vi "getXMLTestSuite.vi"(9 "indent level":i32, 10 "testsuite":T1={"name"="", "errors"=0, "skipped"=0, "tests"=0, "failures"=0, "time"=-1.0, "timestamp"=timestamp(0 s since 1904-01-01), "call-chain"=[], "properties"=variant}, 11 "Test Report in":refnum<class "Test Report.lvclass">) -> (1 "testsuite (end)":string="</testsuite>", 2 "testsuite (start)":string[](array[string]), 3 "Test Report":refnum<class "Test Report.lvclass">)   [LabVIEW 2020, in "Caraya.lvlib" / "Test Report.JUnit.lvclass"]
uses:
  Test Report.JUnit.lvclass
  testsuite -- cluster.ctl
  Test Report/Test Report.lvclass
  MsgSerializer.XML/MsgSerializer.XML.lvclass
  C:/projects/caraya/src/classes/MsgSerializer/MsgSerializer.lvclass
  Test Report/Test Report.lvclass/Test Report.ctl
  MsgSerializer/MsgSerializer.lvclass/MsgSerializer.ctl
  MsgSerializer.XML/format -- enum.ctl
  MsgSerializer.XML/MsgSerializer.XML.lvclass/MsgSerializer.XML.ctl
  MsgSerializer/MsgSerializer.lvclass
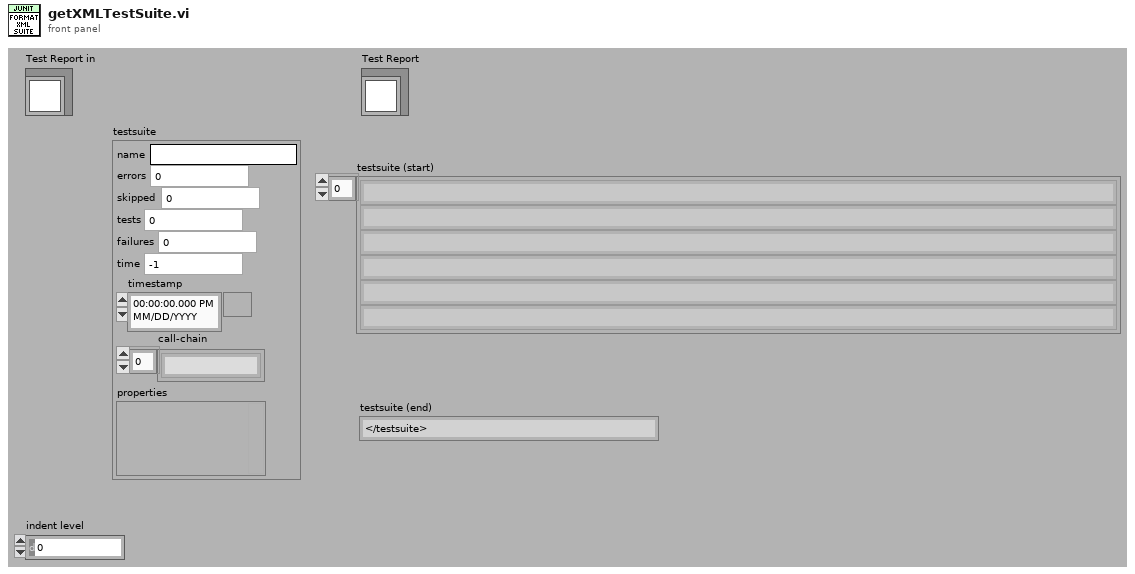
[diagram p1: front panel]
types:
  T1 = typedef "Caraya.lvlib/Test Report.JUnit.lvclass/testsuite -- cluster.ctl" = cluster{"name":string, "errors":u32, "skipped":u32, "tests":u32, "failures":u32, "time":dbl, "timestamp":timestamp, "call-chain":string[], "properties":variant}
  T2 = typedef "Caraya.lvlib/MsgSerializer.XML.lvclass/format -- enum.ctl" = enum16{"value", "tag", "property"}
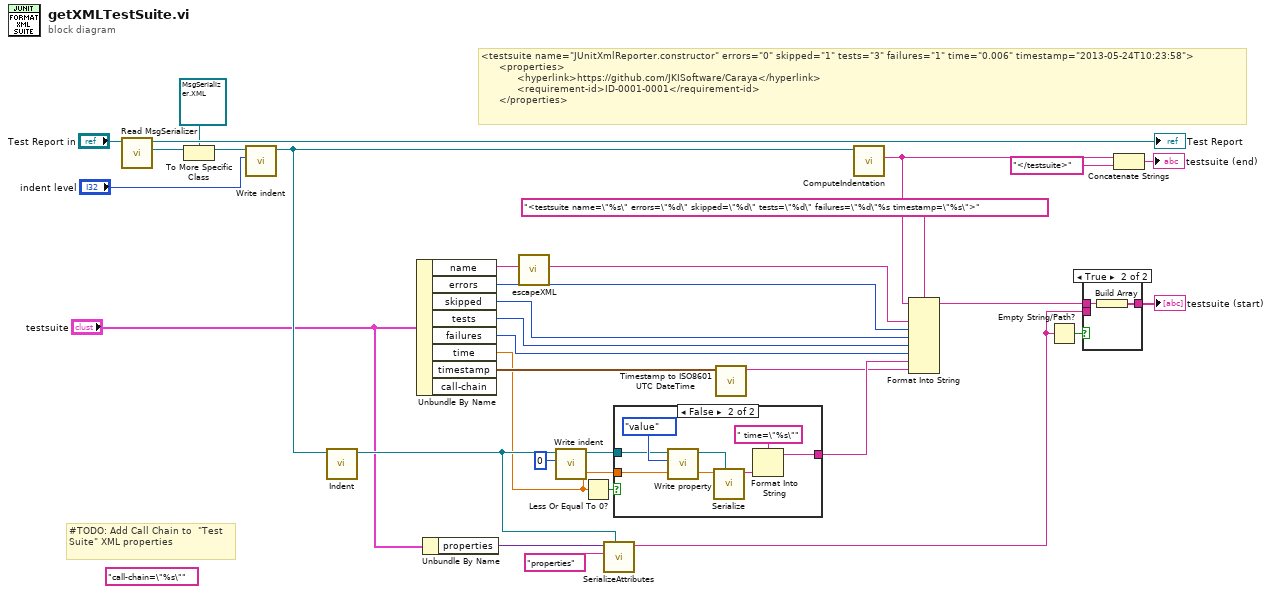
[diagram p0: block diagram]
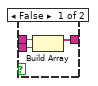
[diagram p3: hidden frame]
diagram:
  (unwired) "call-chain=\"%s\""
  # "#TODO: Add Call Chain to  \"Test Suite\" XML properties"
  # "<testsuite name=\"JUnitXmlReporter.constructor\" errors=\"0\" skipped=\"1\" tests=\"3\" failures=\"1\" time=\"0.006\" timestamp=\"2013-05-24T10:23:58\">\n      <properties>\n            <hyperlink>https://github.com/JKISoftware/Caraya</hyperlink>\n            <requirement-id>ID-0001-0001</requirement-id>\n      </properties>"
  n1 = call "Read MsgSerializer.vi"("Test Report in"="Test Report in") -> ("MsgSerializer"=w2:refnum<class "MsgSerializer.lvclass">, "Test Report out"=→"Test Report":refnum<class "Test Report.lvclass">)  [unwired: 9 in]
  n2 = To More Specific Class(target class=refnum<class "MsgSerializer.XML.lvclass"> refnum ("MsgSerializer"), reference=w2) -> (specific class reference=w1:refnum<class "MsgSerializer.XML.lvclass">)  [unwired: 1 in, 1 out]
  n3 = call "Write indent.vi"("indent"="indent level", "MsgSerializer in"=w1) -> ("MsgSerializer out"=w7:refnum<class "MsgSerializer.XML.lvclass">)  [unwired: 9 in]
  n4 = call "Indent.vi"("MsgSerializer in"=w7) -> ("MsgSerializer out"=w15:refnum<class "MsgSerializer.XML.lvclass">)  [unwired: 10 in]
  n5 = Unbundle By Name("testsuite") -> ("name"=w26:string, "errors"=w32:u32, "skipped"=w31:u32, "tests"=w30:u32, "failures"=w29:u32, "time"=w14:dbl, "timestamp"=w28:timestamp)  [unwired: 1 out]
  n6 = Unbundle By Name("testsuite") -> ("properties"=w9:variant)
  n7 = call "escapeXML.vi"("Input String"=w26) -> ("XML-escaped String"=w25:string)  [unwired: 10 in]
  n8 = call "Write indent.vi"("indent"=0, "MsgSerializer in"=w15) -> ("MsgSerializer out"=w16:refnum<class "MsgSerializer.XML.lvclass">)  [unwired: 9 in]
  n9 = Less Or Equal To 0?(x=w14) -> (x <= 0?=w13:bool)
  n10 = call "SerializeAttributes.vi"("MsgSerializer"=w15, "attribute name"="properties", "variant attribute"=w9) -> ("Serialized Message"=w20:string)  [unwired: 8 in]
  n11 = case shown="False" w13 {
    tunnel: [_ w38] -> w12
    tunnel: w14 -> [_ w37]
    tunnel: w16 -> [_ w34]
    frame True {
    }
    frame False {
      n12 = call "Write property.vi"("format"=format_--_enum."value", "MsgSerializer.XMLProperty in"=w34) -> ("MsgSerializer.XMLProperty out"=w33:refnum<class "MsgSerializer.XML.lvclass">)  [unwired: 9 in]
      n13 = call-dynamic "Serialize.vi"("MsgSerializer"=w33, "Value"=w37) -> ("Serialized Message"=w36:string)  [unwired: 8 in, 1 out]
      n14 = Format Into String(format string=" time=\"%s\"", w36) -> (resulting string=w38:string)  [unwired: 2 in, 1 out]
    }
  }
  n15 = call <vilib>:"Timestamp to ISO8601 UTC DateTime.vi"("Timestamp (now)"=w28) -> ("ISO8601 UTC DateTime"=w10:string)  [unwired: 10 in]
  n16 = call "ComputeIndentation.vi"("MsgSerializer in"=w7) -> ("indentation"=w5:string)  [unwired: 10 in]
  n17 = Format Into String(format string="<testsuite name=\"%s\" errors=\"%d\" skipped=\"%d\" tests=\"%d\" failures=\"%d\"%s timestamp=\"%s\">", initial string=w5, w25, w32, w31, w30, w29, w12, w10) -> (resulting string=w4:string)  [unwired: 1 in, 1 out]
  n18 = Empty String/Path?(string/path=w20) -> (empty?=w21:bool)
  n19 = case shown="True" w21 {
    tunnel: [w42 w43] -> w19
    tunnel: w4 -> [w41 w44]
    tunnel: w20 -> [w40 _]
    frame False {
      n20 = Build Array(w41, w40) -> (w42:string[])
    }
    frame True {
      n21 = Build Array(w44) -> (w43:string[])
    }
  }
  "testsuite (start)" <- w19
  n22 = Concatenate Strings(w5, "</testsuite>" ("testsuite (end)")) -> (→"testsuite (end)":string)
